vi "FuncVI-Beep.vi"(5 "InstanceRef":T2, 9 "arg list":T1[](array[typedef]) {"num" format="%.2f"}) -> (0 "error out":bool, 3 "result":T1 {"num" format="%.2f"})   [LabVIEW 2021]
doc: "::: CalcExpress Toolkit :::\nCopyright (c) 2000-2026 Konstantin Shifershteyn. All rights reserved."
uses:
  cetypes.llb/CalcExpress Function Argument Info.ctl
  cetypes.llb/CalcExpress Instance RefNum.ctl
panel:
  in  "max arg num":i32=2
  in  "min arg num":i32
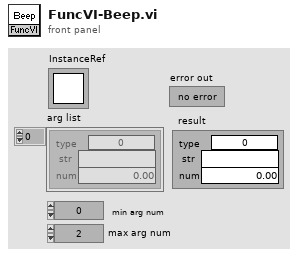
[diagram p1: front panel]
types:
  T1 = typedef "CalcExpress Function Argument Info.ctl" = cluster{"type":u32, "str":string, "num":dbl}
  T2 = typedef "CalcExpress Instance RefNum.ctl" = refnum<k1>
  T3 = cluster{"index":i32, "type":enum8{"String", "DBL Number", "identifier", "1D Array of DBL", "2D Array of DBL", "CDB Number", "1D Array of CDB", "2D Array of CDB", "Unknown data type"}, "default num":dbl, "default str":string}[]
  T4 = enum8{"String", "DBL Number", "identifier", "1D Array of DBL", "2D Array of DBL", "CDB Number", "1D Array of CDB", "2D Array of CDB", "1D Array of String", "2D Array of String", "Unknown data type"}
  T5 = cluster{"type":enum8{"String", "DBL Number", "identifier", "1D Array of DBL", "2D Array of DBL", "CDB Number", "1D Array of CDB", "2D Array of CDB", "1D Array of String", "2D Array of String", "Unknown data type"}, string, "num val":dbl}
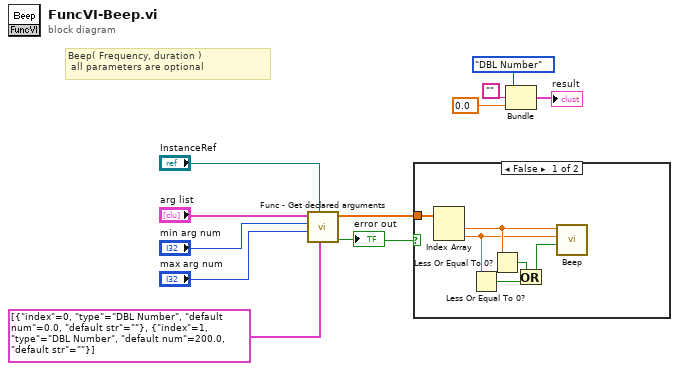
[diagram p0: block diagram]
diagram:
  # "Beep( Frequency, duration ) \n all parameters are optional"
  n1 = call "Func - Get declared arguments.vi"("arg descriptors"=T3 [{"index"=0, "type"=enum."DBL Number", "default num"=0.0, "default str"=""}, {"index"=1, "type"=enum."DBL Number", "default num"=200.0, "default str"=""}] ("args descriptors"), "InstanceRef"="InstanceRef", "max arg num"="max arg num", "min arg num"="min arg num", "arg list"="arg list") -> ("error out"=w10:bool, "num list"=w2:dbl[])  [unwired: 3 in, 2 out]
  "error out" <- w10
  n2 = case shown="False" w10 {
    tunnel: w2 -> [w17 _]
    frame False {
      n3 = Index Array(array=w17) -> (element #1=w16:dbl, element #2=w15:dbl)  [unwired: 2 in]
      n4 = Less Or Equal To 0?(x=w15) -> (x <= 0?=w13:bool)
      n5 = Less Or Equal To 0?(x=w16) -> (x <= 0?=w14:bool)
      n6 = Or(x=w14, y=w13) -> (x .or. y?=w12:bool)
      n7 = call <vilib>:"Beep.vi"("use system alert? (T)"=w12, "duration (msec)"=w15, "frequency (Hz)"=w16) -> ()  [unwired: 9 in]
    }
    frame True {
    }
  }
  n8 = Bundle("type"=T4."DBL Number", "", "num val"=0.0) -> (→"result":T5)  [unwired: 1 in]
